vi "lab2_3_subvi_mem.vi"(8 "Address":u32, 11 "Data In":i16) -> (3 "Last Value":i16)   [LabVIEW 2026]
uses:
  <vilib>/rvi/DataTransferAndStorage/Container/XNode/niFpgaContainer.xnode
  <vilib>/rvi/Memory/Memory_Emulation/nirvimemoryEmulation.vi
  <vilib>/rvi/Memory/Memory_Emulation/nirvimemoryFastEmulation.vi
  <vilib>/rvi/Memory/Memory_Emulation/niFpgaMemoryEmulationRefIn.vi
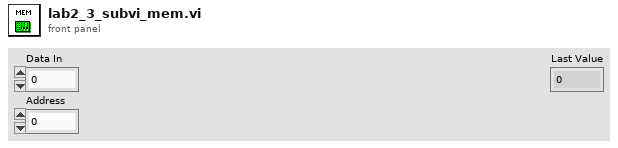
[diagram p1: front panel]
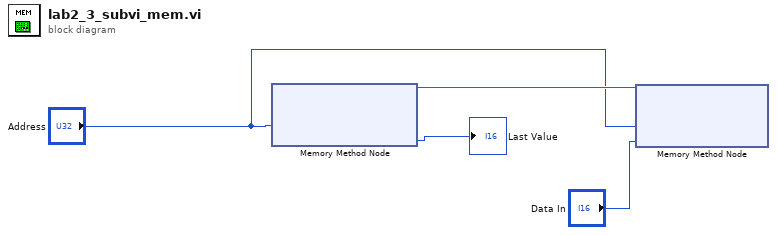
[diagram p0: block diagram]
diagram:
  n1 = xnode ("Memory Method Node")("Address"="Address") -> ("Data"=→"Last Value":i16, "Memory Out"=w4:refnum<k21>)  [unwired: 1 in]
  n2 = xnode ("Memory Method Node")("Address"="Address", "Data"="Data In", "Memory In"=w4) -> ()  [unwired: 1 out]
